vi "set Starting and Num RB.vi"(8 "error in (no error)":errorcluster, 10 "RB Setting Param":T1, 11 "LTE in":refnum<class "LTE.lvclass">) -> (0 "error out":errorcluster, 3 "LTE out":refnum<class "LTE.lvclass">)   [LabVIEW 2023, in "ANRITSU Call Box.lvlib" / "LTE.lvclass"]
uses:
  LTE.lvclass
  LTE.lvclass/LTE.ctl
  Type Definition/LTE RB Setting Params.ctl
  ANRITSU Call Box.lvlib
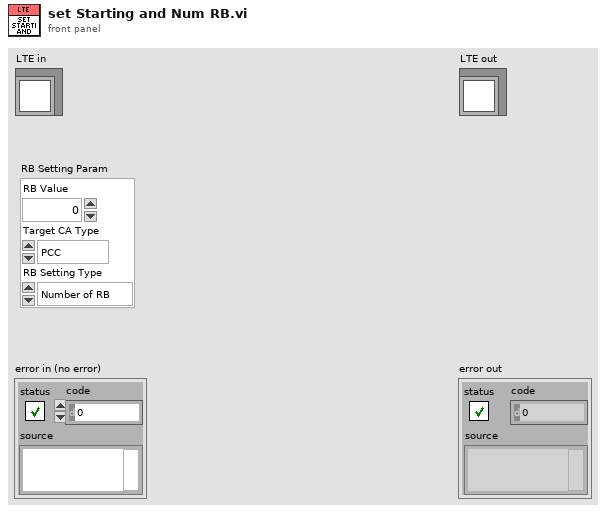
[diagram p1: front panel]
types:
  T1 = typedef "ANRITSU Call Box.lvlib/LTE RB Setting Params.ctl" = cluster{"RB Value":i32, "Target CA Type":enum16{"PCC", "SCC1"}, "RB Setting Type":enum16{"Number of RB", "Starting RB"}}
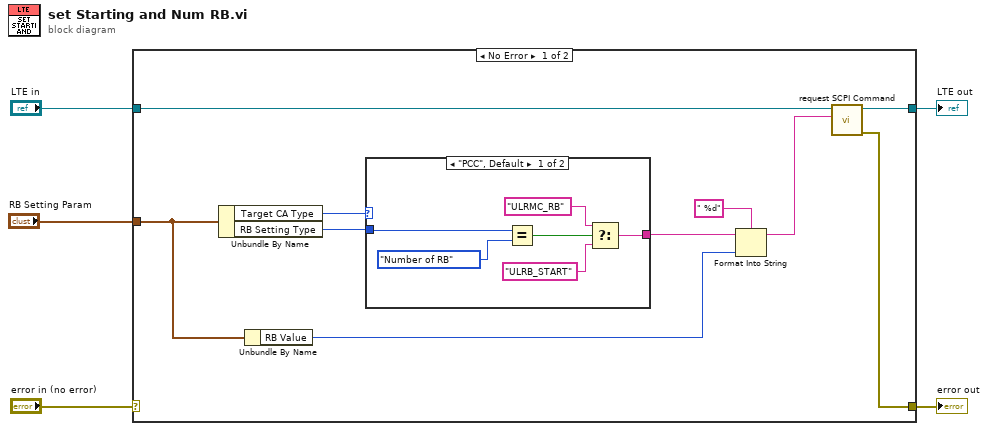
[diagram p0: block diagram]
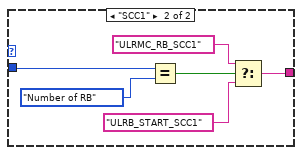
[diagram p2: hidden frame]
diagram:
  n1 = case shown="No Error" "error in (no error)" {
    selector: "error in (no error)" -> [_ w29]
    tunnel: [w6 w29] -> w4
    tunnel: [w8 w28] -> w2
    tunnel: "LTE in" -> [w9 w28]
    tunnel: "RB Setting Param" -> [w11 _]
    frame No Error {
      n2 = Unbundle By Name(w11) -> ("Target CA Type"=w15:enum16{"PCC", "SCC1"}, "RB Setting Type"=w14:enum16{"Number of RB", "Starting RB"})
      n3 = Unbundle By Name(w11) -> ("RB Value"=w10:i32)
      n4 = case shown="\"PCC\", Default" w15 {
        tunnel: w14 -> [w21 w27]
        tunnel: [w16 w22] -> w13
        frame "PCC", Default {
          n5 = Equal?(x=w21, y=enum16{"Number of RB", "Starting RB"}."Number of RB") -> (x = y?=w19:bool)
          n6 = Select(t="ULRMC_RB" ("string"), s=w19, f="ULRB_START" ("string")) -> (s? t:f=w16:string)
        }
        frame "SCC1" {
          n7 = Equal?(x=w27, y=enum16{"Number of RB", "Starting RB"}."Number of RB") -> (x = y?=w25:bool)
          n8 = Select(t="ULRMC_RB_SCC1" ("string"), s=w25, f="ULRB_START_SCC1" ("string")) -> (s? t:f=w22:string)
        }
      }
      n9 = Format Into String(format string=" %d", initial string=w13, w10) -> (resulting string=w7:string)  [unwired: 1 in, 1 out]
      n10 = call "request SCPI Command.vi"("SCPI Command"=w7, "LTE in"=w9) -> ("error out"=w6:errorcluster, "LTE out"=w8:refnum<class "LTE.lvclass">)  [unwired: 8 in]
    }
    frame Error {
    }
  }
  "error out" <- w4
  "LTE out" <- w2
